vi "filterTP.vi"(10 "输入":dbl format="%#_13g") -> (2 "输出":dbl format="%#_13g")   [LabVIEW 2026, in "UI-温度采集.lvlib"]
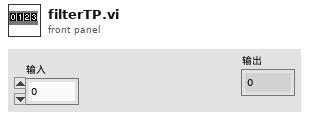
[diagram p1: front panel]
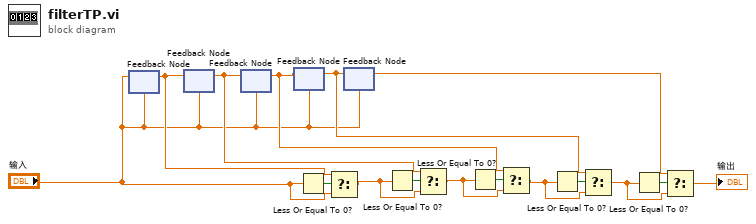
[diagram p0: block diagram]
diagram:
  n1 = feedback #1("输入") -> (w15:dbl)
  n2 = feedback-in #1("输入") -> ()
  n3 = feedback #2("输入") -> (w12:dbl)
  n4 = feedback-in #2(w15) -> ()
  n5 = feedback #3("输入") -> (w9:dbl)
  n6 = feedback-in #3(w12) -> ()
  n7 = feedback #4("输入") -> (w6:dbl)
  n8 = feedback-in #4(w9) -> ()
  n9 = Less Or Equal To 0?(x="输入") -> (x <= 0?=w16:bool)
  n10 = Select(t=w15, s=w16, f="输入") -> (s? t:f=w13:dbl)
  n11 = feedback #5("输入") -> (w3:dbl)
  n12 = feedback-in #5(w6) -> ()
  n13 = Less Or Equal To 0?(x=w13) -> (x <= 0?=w14:bool)
  n14 = Select(t=w12, s=w14, f=w13) -> (s? t:f=w10:dbl)
  n15 = Less Or Equal To 0?(x=w10) -> (x <= 0?=w11:bool)
  n16 = Select(t=w9, s=w11, f=w10) -> (s? t:f=w7:dbl)
  n17 = Less Or Equal To 0?(x=w7) -> (x <= 0?=w8:bool)
  n18 = Select(t=w6, s=w8, f=w7) -> (s? t:f=w4:dbl)
  n19 = Less Or Equal To 0?(x=w4) -> (x <= 0?=w5:bool)
  n20 = Select(t=w3, s=w5, f=w4) -> (s? t:f=→"输出":dbl)
